vi "set Test Channel.vi"(8 "error in (no error)":errorcluster, 9 "Selected CC Argements":T2, 10 "NR Test Channel":T1, 11 "NR in":refnum<class "NR.lvclass">) -> (0 "error out":errorcluster, 3 "NR out":refnum<class "NR.lvclass">)   [LabVIEW 2023, in "ANRITSU Call Box.lvlib" / "NR.lvclass"]
uses:
  NR.lvclass
  NR.lvclass/NR.ctl
  Type Definition/NR Selected CC Type Arguments.ctl
  ANRITSU Call Box.lvlib
  Type Definition/NR Test Channel Type.ctl
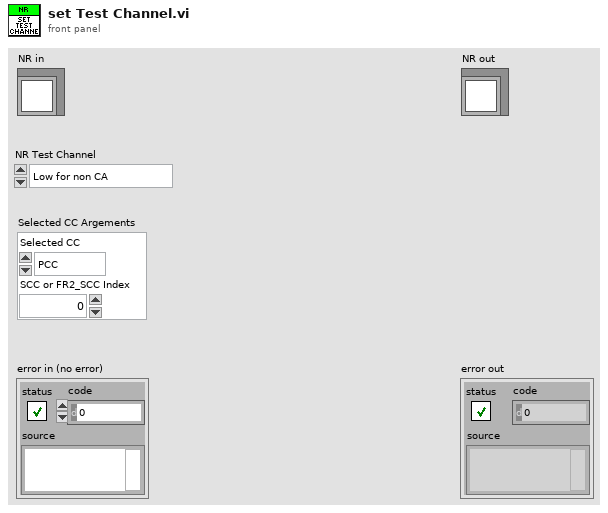
[diagram p1: front panel]
types:
  T1 = typedef "ANRITSU Call Box.lvlib/NR Test Channel Type.ctl" = enum16{"Low for non CA", "Mid for non CA", "High for non CA", "Low for Intra Conti CA", "Mid for Intra Conti CA", "High for Intra Conti CA"}
  T2 = typedef "ANRITSU Call Box.lvlib/NR Selected CC Type Arguments.ctl" = cluster{"Selected CC":enum16{"PCC", "SCC", "FR2_PCC", "FR2_SCC"}, "SCC or FR2_SCC Index":u32}
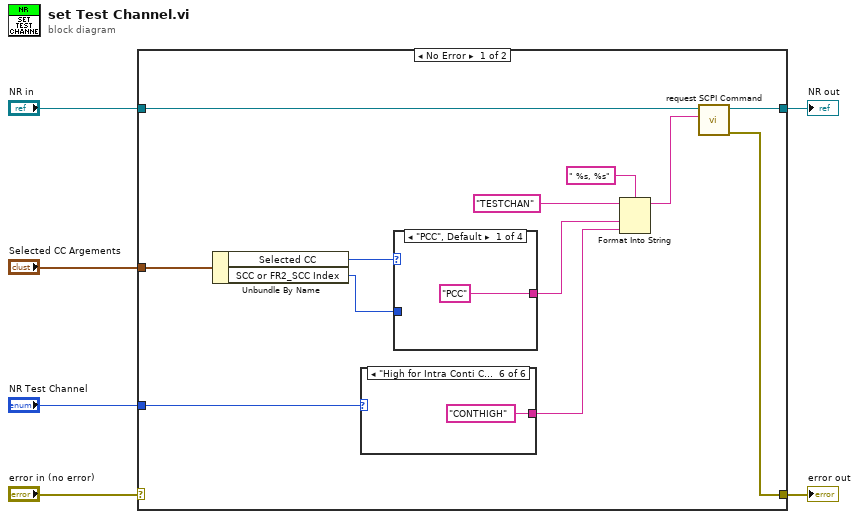
[diagram p0: block diagram]
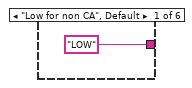
[diagram p2: hidden frame]
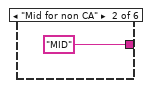
[diagram p3: hidden frame]
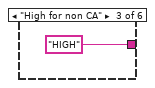
[diagram p4: hidden frame]
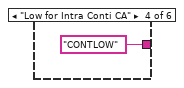
[diagram p5: hidden frame]
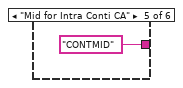
[diagram p6: hidden frame]
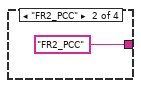
[diagram p7: hidden frame]
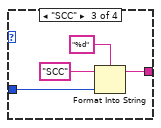
[diagram p8: hidden frame]
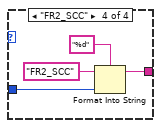
[diagram p9: hidden frame]
diagram:
  n1 = case shown="No Error" "error in (no error)" {
    selector: "error in (no error)" -> [_ w36]
    tunnel: [w7 w36] -> w5
    tunnel: [w9 w35] -> w3
    tunnel: "NR in" -> [w10 w35]
    tunnel: "Selected CC Argements" -> [w18 _]
    tunnel: "NR Test Channel" -> [w12 _]
    frame No Error {
      n2 = Unbundle By Name(w18) -> ("Selected CC"=w17:enum16{"PCC", "SCC", "FR2_PCC", "FR2_SCC"}, "SCC or FR2_SCC Index"=w16:u32)
      n3 = case shown="\"High for Intra Conti CA\"" w12 {
        tunnel: ["LOW" "MID" "HIGH" "CONTLOW" "CONTMID" "CONTHIGH"] -> w11
        frame "Low for non CA", Default {
        }
        frame "Mid for non CA" {
        }
        frame "High for non CA" {
        }
        frame "Low for Intra Conti CA" {
        }
        frame "Mid for Intra Conti CA" {
        }
        frame "High for Intra Conti CA" {
        }
      }
      n4 = case shown="\"PCC\", Default" w17 {
        tunnel: ["PCC" "FR2_PCC" w27 w31] -> w13
        tunnel: w16 -> [_ _ w28 w32]
        frame "PCC", Default {
        }
        frame "FR2_PCC" {
        }
        frame "SCC" {
          n5 = Format Into String(format string="%d", initial string="SCC", w28) -> (resulting string=w27:string)  [unwired: 1 in, 1 out]
        }
        frame "FR2_SCC" {
          n6 = Format Into String(format string="%d", initial string="FR2_SCC", w32) -> (resulting string=w31:string)  [unwired: 1 in, 1 out]
        }
      }
      n7 = Format Into String(format string=" %s, %s", initial string="TESTCHAN", w13, w11) -> (resulting string=w8:string)  [unwired: 1 in, 1 out]
      n8 = call "request SCPI Command.vi"("SCPI Command"=w8, "NR in"=w10) -> ("error out"=w7:errorcluster, "NR out"=w9:refnum<class "NR.lvclass">)  [unwired: 8 in]
    }
    frame Error {
    }
  }
  "error out" <- w5
  "NR out" <- w3
